vi "Add Update Node.vi"(8 "error in (no error)":errorcluster, 10 "Assertion":refnum<class "TestManagerMsg.Assertion.lvclass">, 11 "Test Event Storage in":refnum<class "Test Event Storage.lvclass">) -> (0 "error out":errorcluster, 1 "Test ID":string, 3 "Test Event Storage out":refnum<class "Test Event Storage.lvclass">)   [LabVIEW 2020, in "Caraya.lvlib" / "Test Event Storage.lvclass"]
uses:
  Test Event Storage.lvclass
  Test Manager Message Assertion/TestManagerMsg.Assertion.lvclass
  C:/projects/caraya/src/classes/Test Manager Message/TestManagerMsg.lvclass
  Test Event Storage.lvclass/Test Event Storage.ctl
  Test Manager Message/TestManagerMsg.lvclass/TestManagerMsg.ctl
  test store -- cluster.ctl
  Test Manager Message Test/TestManagerMsg.Test.lvclass
  Test Manager Message/TestManagerMsg.lvclass
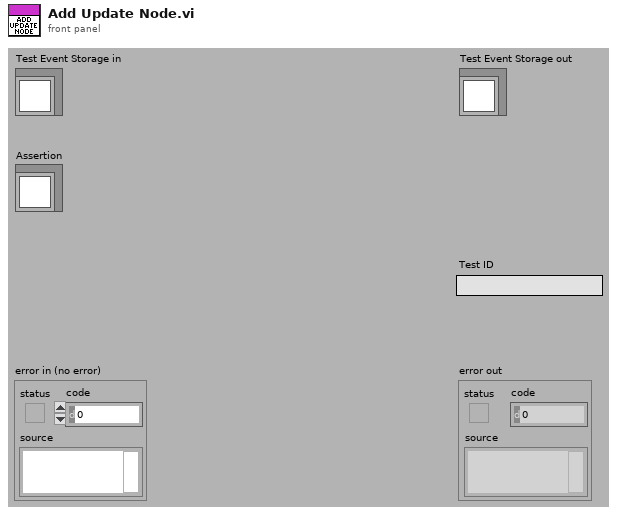
[diagram p1: front panel]
types:
  T1 = typedef "Caraya.lvlib/Test Event Storage.lvclass/test store -- cluster.ctl" = cluster{"Test":refnum<class "TestManagerMsg.Test.lvclass">, "Defined":bool, "Passed":bool, "properties":variant, "assert-ids":variant}
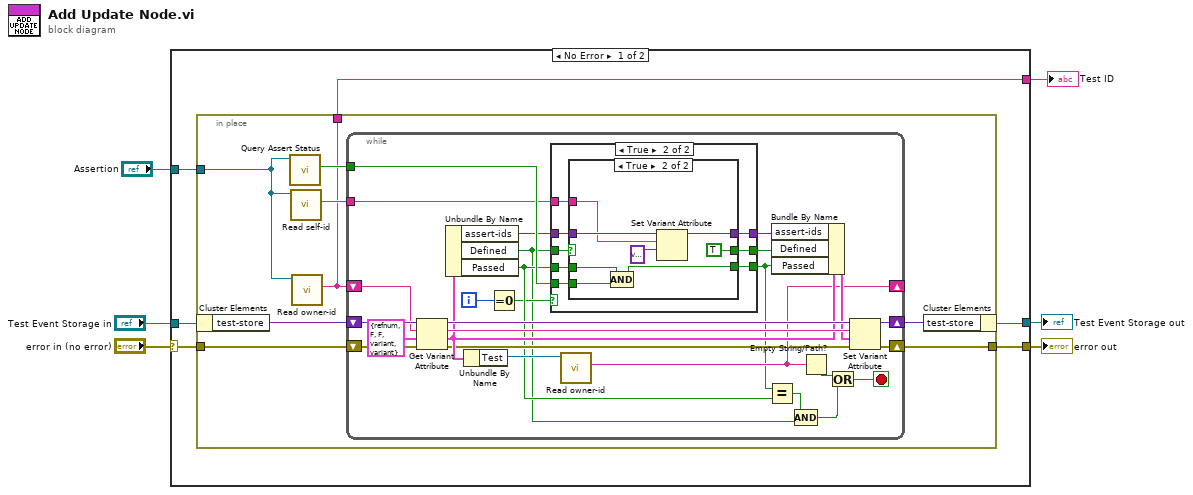
[diagram p0: block diagram]
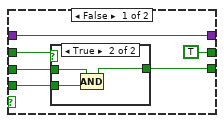
[diagram p2: hidden frame]
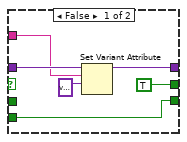
[diagram p4: hidden frame]
diagram:
  n1 = case shown="No Error" "error in (no error)" {
    selector: "error in (no error)" -> [w12 w80]
    tunnel: [w11 w80] -> w5
    tunnel: [w10 w79] -> w4
    tunnel: "Test Event Storage in" -> [w8 w79]
    tunnel: [w9 _] -> w3
    tunnel: "Assertion" -> [w7 _]
    frame No Error {
      n2 = in-place {
        in-place-border: w7 -> [w17]
        in-place-border: [w15] -> w9
        in-place-border: w12 -> [w14]
        in-place-border: [w13] -> w11
        n3 = in-place-cluster #1(w8) -> ("test-store"=w18:variant)
        n4 = call "Query Assert Status.vi"("TestManagerMsg.Assertion in"=w17) -> ("Passed"=w19:bool)  [unwired: 7 in, 3 out]
        n5 = call "Read self-id.vi"("TestManagerMsg in"=w17) -> ("self-id"=w20:string)  [unwired: 9 in, 1 out]
        n6 = call "Read owner-id.vi"("TestManagerMsg in"=w17) -> ("owner-id"=w15:string)  [unwired: 9 in, 1 out]
        n7 = while {
          tunnel: w19 -> [w40]
          shift-right: [w37] -> w16
          shift-left: w18 -> [w46]
          tunnel: w20 -> [w35]
          shift-right: [w34] -> _
          shift-left: w15 -> [w42]
          shift-right: [w31] -> w13
          shift-left: w14 -> [w33]
          i -> [w36]
          stop <- w29 stop-if-true
          n8 = Get Variant Attribute(Variant=w46, name=w42, default value (empty Variant)=T1 {"Test"=refnum, "Defined"=FALSE, "Passed"=FALSE, "properties"=variant, "assert-ids"=variant} ("test-store"), error in=w33) -> (duplicate Variant=w43:variant, value=w39:T1, error out=w32:errorcluster)  [unwired: 1 out]
          n9 = Unbundle By Name(w39) -> ("assert-ids"=w26:variant, "Defined"=w21:bool, "Passed"=w27:bool)
          n10 = Unbundle By Name(w39) -> ("Test"=w38:refnum<class "TestManagerMsg.Test.lvclass">)
          n11 = Equal To 0?(x=w36) -> (x = 0?=w23:bool)
          n12 = case shown="True" w23 {
            tunnel: w21 -> [w48 w64]
            tunnel: [TRUE w63] -> w44
            tunnel: [w50 w62] -> w28
            tunnel: w27 -> [w52 w61]
            tunnel: w40 -> [w51 w60]
            tunnel: w35 -> [_ w59]
            tunnel: w26 -> [w47 w58]
            tunnel: [w47 w57] -> w25
            frame False {
              n13 = case shown="True" w48 {
                tunnel: w52 -> [_ w56]
                tunnel: w51 -> [w53 w55]
                tunnel: [w53 w54] -> w50
                frame False {
                }
                frame True {
                  n14 = Compound Arithmetic op=AND(w56, w55) -> (w54:bool)
                }
              }
            }
            frame True {
              n15 = case shown="True" w64 {
                tunnel: w59 -> [w66 w73]
                tunnel: [TRUE TRUE] -> w63
                tunnel: [w69 w77] -> w62
                tunnel: w61 -> [_ w78]
                tunnel: w60 -> [w69 w76]
                tunnel: w58 -> [w68 w74]
                tunnel: [w67 w72] -> w57
                frame False {
                  n16 = Set Variant Attribute(Variant=w68, name=w66, value=variant ("variant")) -> (Variant out=w67:variant)  [unwired: 1 in, 2 out]
                }
                frame True {
                  n17 = Compound Arithmetic op=AND(w78, w76) -> (w77:bool)
                  n18 = Set Variant Attribute(Variant=w74, name=w73, value=variant ("variant")) -> (Variant out=w72:variant)  [unwired: 1 in, 2 out]
                }
              }
            }
          }
          n19 = call "Read owner-id.vi"("TestManagerMsg in"=w38) -> ("owner-id"=w34:string)  [unwired: 9 in, 1 out]
          n20 = Equal?(x=w28, y=w27) -> (x = y?=w24:bool)
          n21 = Bundle By Name(cluster=w39, "assert-ids"=w25, "Defined"=w44, "Passed"=w28) -> (w41:T1)
          n22 = Compound Arithmetic op=AND(w24, w21) -> (w22:bool)
          n23 = Empty String/Path?(string/path=w34) -> (empty?=w30:bool)
          n24 = Or(x=w30, y=w22) -> (x .or. y?=w29:bool)
          n25 = Set Variant Attribute(Variant=w43, name=w42, value=w41, error in=w32) -> (Variant out=w37:variant, error out=w31:errorcluster)  [unwired: 1 out]
        }
        n26 = in-place-cluster #1("test-store"=w16) -> (w10:refnum<class "Test Event Storage.lvclass">)
      }
    }
    frame Error {
    }
  }
  "error out" <- w5
  "Test Event Storage out" <- w4
  "Test ID" <- w3
